vi "Constants.vi"() -> ()   [LabVIEW 2025, in "Keithley-DAQ6510 Shared.lvlib"]
doc: "Use this Global VI to access the GUIDs assigned to the page resources of the Custom Device."
uses:
  Keithley-DAQ6510 Shared.lvlib
panel:
  in  "Tab Control":enum32{"GUIDs", "Constants", "Properties"}(tab)
  in  "Keithley-DAQ6510":string="303bfb56-379a-4296-9cfb-9ed7b6af0f0a"
  in  "Compiled.Settings":string="Compiled.Settings"
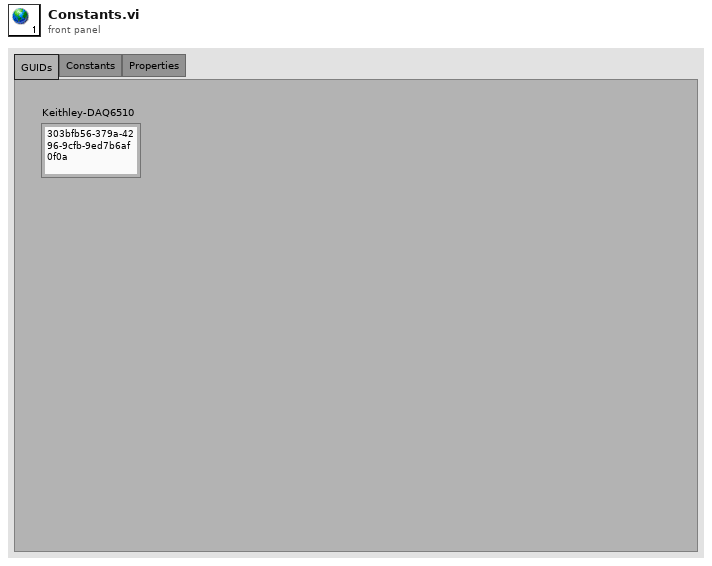
[diagram p1: front panel]
diagram:
